vi "XPN Set Calibration Directory.vi"(8 "error in (no error)":errorcluster, 11 "dirPath":string) -> (0 "error out":errorcluster, 3 "function return":i32)   [LabVIEW 2022 SP3, in "xPanelWrapper.lvlib"]
doc: "XPN_API int XPN_SetCalibrationDirectory(const char* dirPath);"
uses:
  xPanelWrapper.lvlib
  xPanelWrapper.dll
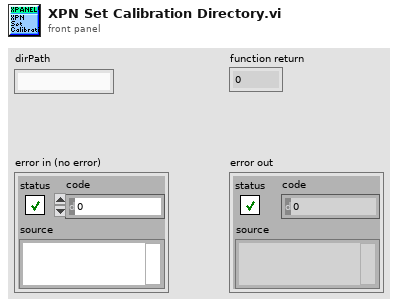
[diagram p1: front panel]
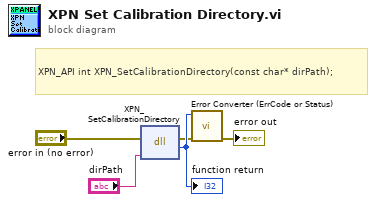
[diagram p0: block diagram]
diagram:
  # "XPN_API int XPN_SetCalibrationDirectory(const char* dirPath);"
  n1 = dll-call lib="E:/SourceCodes/image-harvest/ImageHandler/xPanelWrapperLvLib/xPanelWrapper.*" fn="XPN_SetCalibrationDirectory"(error in="error in (no error)", "dirPath"="dirPath") -> (error out=w2:errorcluster, w5:i32)  [unwired: 3 in, 1 out]
  "function return" <- w5
  n2 = call "Error Converter (ErrCode or Status).vi"("error in (no error)"=w2, "error code"=w5) -> ("error out"=→"error out":errorcluster)  [unwired: 9 in]
